vi "Read File.vi"(9 "文件参数":T1={"时间列"=1, "名称行"=4, "单位行"=4, "数据首行"=5, "数据首列"=2, "分隔符"=enum."逗号"}, 10 "File Type":T3, 11 "Path":path=path "D:/同步空间/曲线生成/原始曲线/1-1、伟思1 原始数据 --mande.x66") -> (1 "Data Series":T2[](array[typedef]))   [LabVIEW 2020, in "Data Viewer.lvlib"]
uses:
  Data Viewer.lvlib
  File Type--enum.ctl
  Data Serie--cluster.ctl
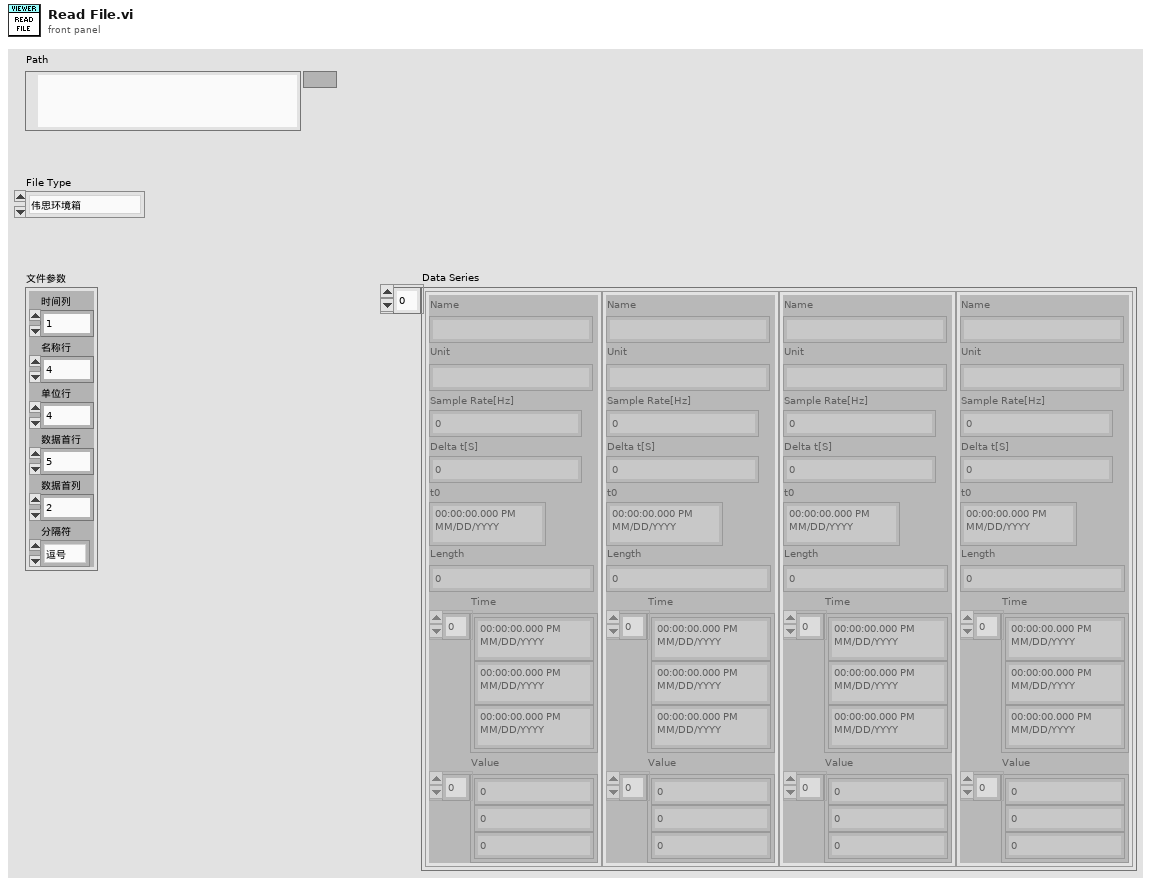
[diagram p1: front panel]
types:
  T1 = cluster{"时间列":i32, "名称行":i32, "单位行":i32, "数据首行":i32, "数据首列":i32, "分隔符":enum16{"逗号", "制表符"}}
  T2 = typedef "Data Viewer.lvlib/Data Serie--cluster.ctl" = cluster{"Name":string, "Unit":string, "Sample Rate[Hz]":dbl, "Delta t[S]":dbl, "t0":timestamp, "Length":i32, "Time":timestamp[], "Value":dbl[]}
  T3 = typedef "Data Viewer.lvlib/File Type--enum.ctl" = enum16{"伟思环境箱", "增达环境箱", "广五所环境箱", "无纸记录仪", "帕捷SA00339", "记录仪840", "记录仪8400", "记录仪MR888", "*.csv"}
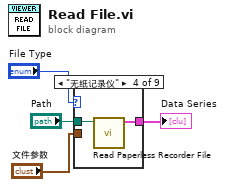
[diagram p0: block diagram]
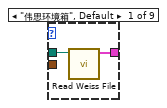
[diagram p2: hidden frame]
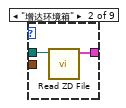
[diagram p3: hidden frame]
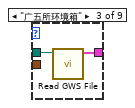
[diagram p4: hidden frame]
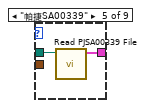
[diagram p5: hidden frame]
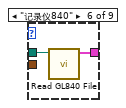
[diagram p6: hidden frame]
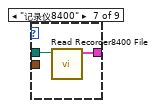
[diagram p7: hidden frame]
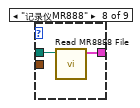
[diagram p8: hidden frame]
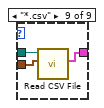
[diagram p9: hidden frame]
diagram:
  n1 = case shown="\"无纸记录仪\"" "File Type" {
    tunnel: "Path" -> [w6 w8 w10 w12 w14 w16 w18 w20 w23]
    tunnel: [w5 w7 w9 w11 w13 w15 w17 w19 w21] -> w2
    tunnel: "文件参数" -> [_ _ _ _ _ _ _ _ w22]
    frame "伟思环境箱", Default {
      n2 = call "Read Weiss File.vi"("Path"=w6) -> ("Data Series"=w5:T2[])  [unwired: 10 in]
    }
    frame "增达环境箱" {
      n3 = call "Read ZD File.vi"("Path"=w8) -> ("Data Series"=w7:T2[])  [unwired: 10 in]
    }
    frame "广五所环境箱" {
      n4 = call "Read GWS File.vi"("Path"=w10) -> ("Data Series"=w9:T2[])  [unwired: 10 in]
    }
    frame "无纸记录仪" {
      n5 = call "Read Paperless Recorder File.vi"("Path"=w12) -> ("Data Series"=w11:T2[])  [unwired: 10 in]
    }
    frame "帕捷SA00339" {
      n6 = call "Read PJSA00339 File.vi"("Path"=w14) -> ("Data Series"=w13:T2[])  [unwired: 10 in]
    }
    frame "记录仪840" {
      n7 = call "Read GL840 File.vi"("Path"=w16) -> ("Data Series"=w15:T2[])  [unwired: 10 in]
    }
    frame "记录仪8400" {
      n8 = call "Read Recorder8400 File.vi"("Path"=w18) -> ("Data Series"=w17:T2[])  [unwired: 10 in]
    }
    frame "记录仪MR888" {
      n9 = call "Read MR8888 File.vi"("Path"=w20) -> ("Data Series"=w19:T2[])  [unwired: 10 in]
    }
    frame "*.csv" {
      n10 = call "Read CSV File.vi"("文件参数"=w22, "Path"=w23) -> ("Data Series"=w21:T2[])  [unwired: 9 in]
    }
  }
  "Data Series" <- w2
